vi "XMLTrustClientCertification.vi"(8 "Error In":errorcluster, 10 "OPC UA server refnum in":refnum<k21>, 11 "DOM document in":refnum<k20>) -> (0 "Error Out":errorcluster, 1 "trusted client certfications":path[](array[path]), 2 "OPC UA server refnum out":refnum<k21>, 3 "DOM document out":refnum<k20>)   [LabVIEW 2014, in "OPCUA XML(dev).lvlib"]
uses:
  OPCUA XML(dev).lvlib
  <resource>/objmgr/DOMUserDefRef.rc
  <vilib>/xml/NI_XML.lvlib
  <vilib>/xml/Close Reference(Node).vi
  <vilib>/OPCUA/NI OPC UA Server.lvlib
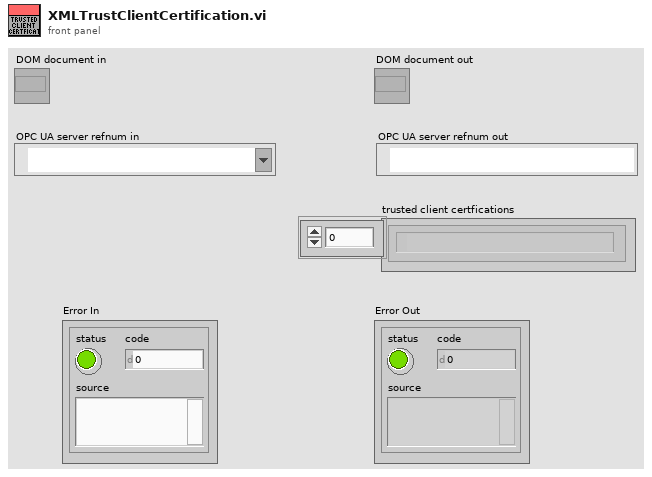
[diagram p1: front panel]
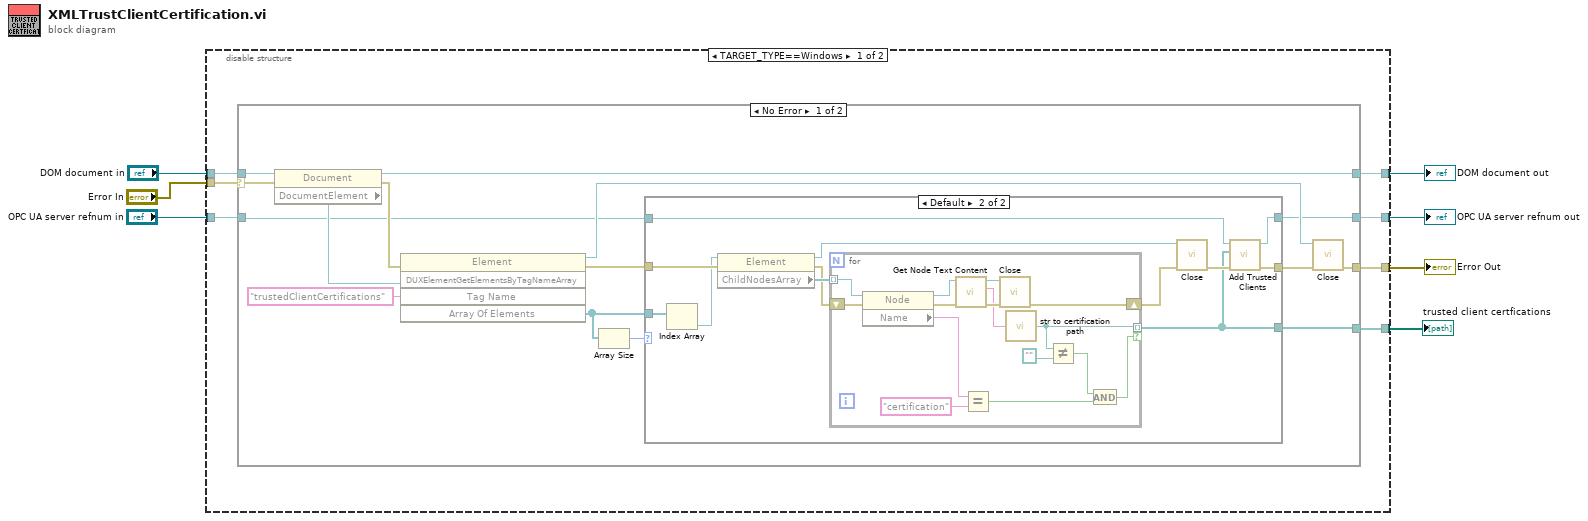
[diagram p0: block diagram]
diagram:
  n1 = disable-structure shown="TARGET_TYPE==Windows" {
    disable-tunnel: [w14 w63] -> w7
    disable-tunnel: "Error In" -> [w13 w63]
    disable-tunnel: "DOM document in" -> [w12 w62]
    disable-tunnel: [w11 w62] -> w4
    disable-tunnel: [w10 _] -> w3
    disable-tunnel: "OPC UA server refnum in" -> [w9 _]
    disable-tunnel: [w8 _] -> w1
    frame condition #0 {
      n2 = case shown="No Error" w13 {
        selector: w13 -> [w29 w61]
        tunnel: [w26 w61] -> w14
        tunnel: w12 -> [w28 w60]
        tunnel: [w27 w60] -> w11
        tunnel: [w17 w59] -> w10
        tunnel: w9 -> [w16 w59]
        tunnel: [w15 _] -> w8
        frame No Error {
          n3 = property class="Document"(reference=w28, error in=w29) -> (reference out=w27:refnum<k20>, error out=w21:errorcluster, "DocumentElement"=w23:refnum<k20>)
          n4 = invoke class="Element" method="DUXElementGetElementsByTagNameArray"(reference=w23, error in=w21, "Tag Name"="trustedClientCertifications") -> (reference out=w20:refnum<k20>, error out=w24:errorcluster, "Array Of Elements"=w19:refnum<k20>[])  [unwired: 2 in, 2 out]
          n5 = Array Size(array=w19) -> (size(s)=w18:i32)
          n6 = case shown="Default" w18 {
            tunnel: [w31 w35] -> w25
            tunnel: w24 -> [w31 w43]
            tunnel: w19 -> [_ w38]
            tunnel: [w30 w34] -> w17
            tunnel: w16 -> [w30 w33]
            tunnel: [_ w32] -> w15
            frame 0 {
            }
            frame Default {
              n7 = Index Array(array=w38) -> (element=w37:refnum<k20>)  [unwired: 1 in]
              n8 = property class="Element"(reference=w37, error in=w43) -> (reference out=w42:refnum<k20>, error out=w40:errorcluster, "ChildNodesArray"=w41:refnum<k20>[])
              n9 = for {
                tunnel: w41 -> [w55] mode=indexing
                tunnel: [w47] -> w32 mode=indexing if=w45
                shift-right: [w56] -> w39
                shift-left: w40 -> [w54]
                n10 = property class="Node"(reference=w55, error in=w54) -> (reference out=w53:refnum<k20>, error out=w49:errorcluster, "Name"=w52:string)
                n11 = call <vilib>:"Get Node Text Content.vi"("error in (no error)"=w49, "node in"=w53) -> ("error out"=w58:errorcluster, "node text"=w48:string, "node out"=w57:refnum<k20>)  [unwired: 7 out]
                n12 = Equal?(x=w52, y="certification") -> (x = y?=w50:bool)
                n13 = call-poly <vilib>:"Close.vi"("error in (no error)"=w58, "node"=w57) -> ("error out"=w56:errorcluster)  [unwired: 7 out]
                n14 = call "str to certification path.vi"("node text"=w48) -> ("File Path Control"=w47:path)  [unwired: 4 in]
                n15 = Not Equal?(x=w47, y=path "") -> (x != y?=w44:bool)
                n16 = And(x=w44, y=w50) -> (x .and. y?=w45:bool)
              }
              n17 = call-poly <vilib>:"Close.vi"("error in (no error)"=w39, "node"=w42) -> ("error out"=w36:errorcluster)  [unwired: 7 out]
              n18 = call <vilib>:"Add Trusted Clients.vi"("error in (no error)"=w36, "trusted client certificates"=w32, "OPC UA server refnum in"=w33) -> ("error out"=w35:errorcluster, "OPC UA server refnum out"=w34:refnum<k21>)  [unwired: 7 in]
            }
          }
          n19 = call-poly <vilib>:"Close.vi"("error in (no error)"=w25, "node"=w20) -> ("error out"=w26:errorcluster)  [unwired: 7 out]
        }
        frame Error {
        }
      }
    }
    frame condition #1 (active) {
    }
  }
  "Error Out" <- w7
  "DOM document out" <- w4
  "OPC UA server refnum out" <- w3
  "trusted client certfications" <- w1
